vi "Get Subpanel Status.vi"(0 "GUI Container in":refnum<class "GUI Container.lvclass">, 7 "Subpanel":string, 11 "error in (no error)":errorcluster) -> (4 "GUI Container out":refnum<class "GUI Container.lvclass">, 6 "Subpanel Status":T1, 8 "Subpanel Found":bool, 15 "error out":errorcluster)   [LabVIEW 2023, in "GUI Views.lvlib" / "GUI Container.lvclass"]
uses:
  GUI Container.lvclass
  typedefs/Subpanel Status.ctl
  GUI Container.lvclass/GUI Container.ctl
  <vilib>/Utility/error.llb/Error Cluster From Error Code.vi
  <vilib>/ErrorRing/Error Ring.xnode
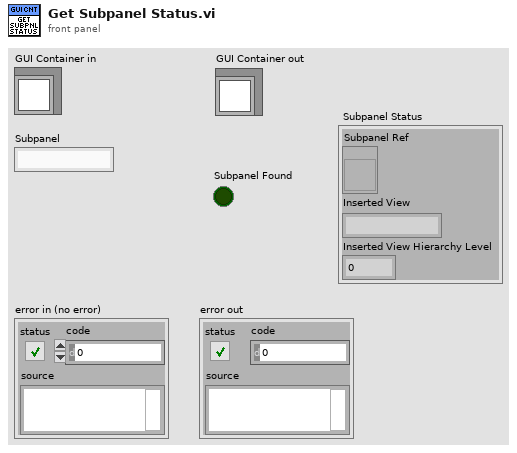
[diagram p1: front panel]
types:
  T1 = typedef "GUI Views.lvlib/GUI Container.lvclass/Subpanel Status.ctl" = cluster{"Subpanel Ref":refnum<vi>, "Inserted View":string, "Inserted View Hierarchy Level":i32}
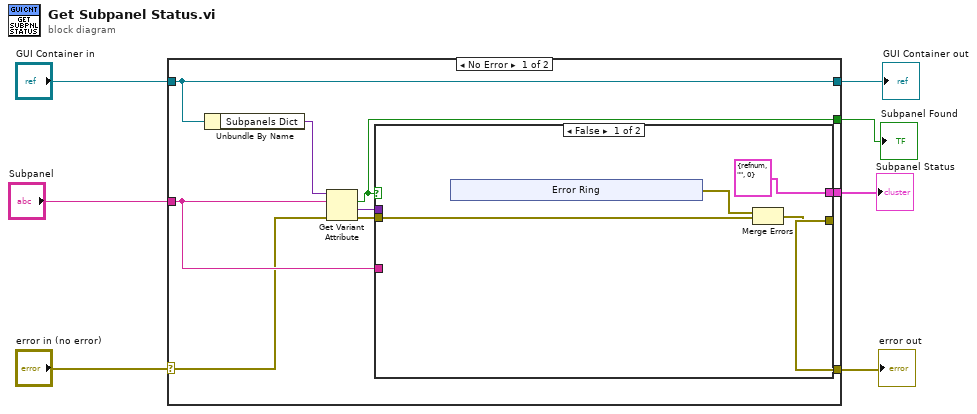
[diagram p0: block diagram]
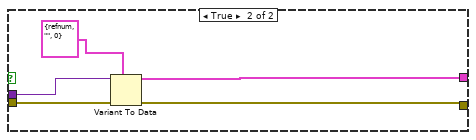
[diagram p2: hidden frame]
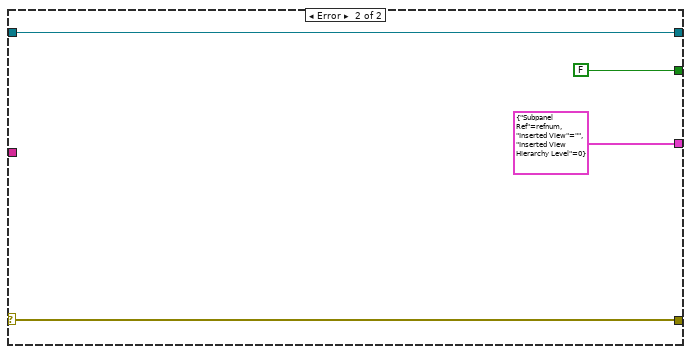
[diagram p3: hidden frame]
diagram:
  n1 = case shown="No Error" "error in (no error)" {
    selector: "error in (no error)" -> [w13 w32]
    tunnel: [w16 w32] -> w7
    tunnel: "GUI Container in" -> [w14 w33]
    tunnel: "Subpanel" -> [w15 _]
    tunnel: [w14 w33] -> w3
    tunnel: [w9 T1 {"Subpanel Ref"=refnum, "Inserted View"="", "Inserted View Hierarchy Level"=0} ("Subpanel Status")] -> w2
    tunnel: [w8 FALSE] -> w1
    frame No Error {
      n2 = Unbundle By Name(w14) -> ("Subpanels Dict"=w12:variant)
      n3 = Get Variant Attribute(Variant=w12, name=w15, error in=w13) -> (found=w8:bool, value=w10:variant, error out=w11:errorcluster)  [unwired: 1 in, 1 out]
      n4 = case shown="False" w8 {
        tunnel: w11 -> [w19 w29]
        tunnel: w10 -> [_ w28]
        tunnel: [w18 w27] -> w16
        tunnel: w15 -> [_ _]
        tunnel: [T1 {"Subpanel Ref"=refnum, "Inserted View"="", "Inserted View Hierarchy Level"=0} ("Subpanel Status") w26] -> w9
        frame False {
          n5 = xnode "Error Ring"() -> ("error out"=w17:errorcluster)
          n6 = Merge Errors(w17, w19) -> (w18:errorcluster)
        }
        frame True {
          n7 = Variant To Data(error in=w29, type=T1 {"Subpanel Ref"=refnum, "Inserted View"="", "Inserted View Hierarchy Level"=0} ("Subpanel Status"), Variant=w28) -> (data=w26:T1, error out=w27:errorcluster)
        }
      }
    }
    frame Error {
    }
  }
  "error out" <- w7
  "GUI Container out" <- w3
  "Subpanel Found" <- w1
  "Subpanel Status" <- w2
